vi "MQTT Client - Configure Auth.vi"(0 "MQTT Session":T1, 5 "Client ID":string, 7 "Username":string, 9 "Password":string, 11 "error in (no error)":errorcluster) -> (4 "MQTT Session out":T1, 15 "error out":errorcluster)   [LabVIEW 2019, in "KoRE-MQTT.lvlib"]
doc: "<b>Description:</b> This VI configures authentication settings for an MQTT client session. It processes client identification information necessary for establishing user authentication with the MQTT broker.\n\n<b>Input Terminals:</b>\n- <b>MQTT Session [0]</b>: Reference to the MQTT session that will utilize the configured authentication settings.\n- <b>Client ID [5]</b>: Unique identifier for the MQTT client, which establishes its identity when communicating with the broker. A pseudo-random Client ID will be generated if this input terminal is not wired.\n- <b>Username [7]</b>: The username required for authenticating with the MQTT broker. Do not wire this input terminal if you intend to connect anonymously to the MQTT broker but are using this VI to set the Client ID.\n- <b>Password [9]</b>: The password corresponding to the provided username, crucial for the authentication process. This terminal must be wired if the Username terminal is connected.\n\n<b>Output Terminals:</b>\n- <b>MQTT Session out [4]</b>: Reference to the configured MQTT session with the applied authentication settings.\n\n\nCopyright (c) 2025 KoRElibs.com\nSPDX-License-Identifier: EUPL-1.2\n\nThis VI is licensed under the European Union Public License (EUPL) Version 1.2. You may use this VI unmodified in proprietary works. If you distribute a modified version of this file, the modified file must be released under the EUPL-1.2. Full license: https://joinup.ec.europa.eu/asset/eupl/eupl/1.2/"
uses:
  KoRE-MQTT.lvlib
  TypeDefs/MQTT Client Session.ctl
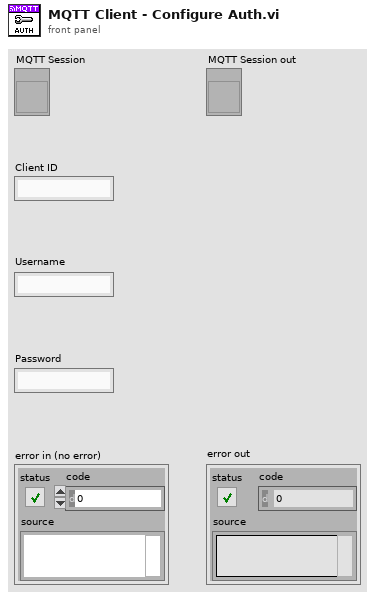
[diagram p1: front panel]
types:
  T1 = typedef "KoRE-MQTT.lvlib/MQTT Client Session.ctl" = refnum<vi>
  T2 = typedef "KoRE-MQTT.lvlib/MQTT Client Session - Data.ctl" = cluster{"TCP ref":refnum<k5>, "Next Packet Id":u16, "Version":u8, "Host":string, "Port":u16, "Ping Delta":u32, "Username":string, "Password":string, "Will QoS":u8, "Will Retain":bool, "Will Topic":string, "Will Payload":string, "TCP Timeout":i32, "Semaphore":T3, "In-Flight Messages":variant, "Close":bool, "Last Send":u32, "Keep Alive":u16, "Last Ping RTT":u32, "Last Ping":u32, "Will Properties":T4[], "Session Expiry Interval":u32, "Maximum QoS":u8, "Retain Available":bool, "Server Maximum Packet Size":u32, "Client Identifier":string, "Server Topic Alias Maximum":u16, "Wildcard Subscription Available":bool, "Subscription Identifier Available":bool, "Shared Subscription Available":bool, "Connect Properties":T5[], "Client Maximum Packet Size":u32, "Client Topic Alias Maximum":u16, "Server Receive Maximum":u16, "Client Receive Maximum":u16, "TLS cfg":refnum<k36>, "Subscriptions":T6[]}
  T3 = typedef "Semaphore RefNum" = refnum<k1>
  T4 = typedef "KoRE-MQTT.lvlib/MQTT Property - Will.ctl" = cluster{"Property":u8, "Value":string}
  T5 = typedef "KoRE-MQTT.lvlib/MQTT Property - CONNECT.ctl" = cluster{"Property":u8, "Value":string}
  T6 = typedef "KoRE-MQTT.lvlib/MQTT Subscription - Info.ctl" = cluster{"Packet Id":u16, "Index":u16, "Identifier":u32, "QoS":u8, "Topic Filter":string, "Reason Code":u8, "Reason String":string, "Granted":bool}
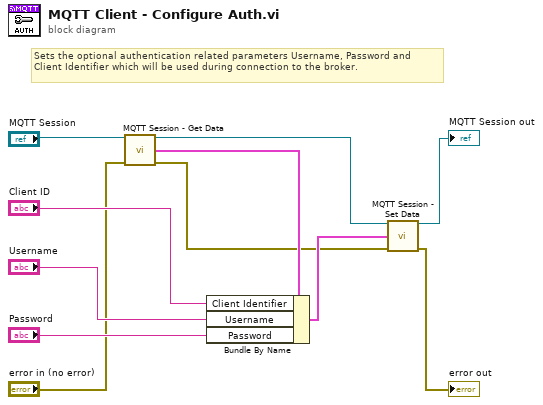
[diagram p0: block diagram]
diagram:
  # "Sets the optional authentication related parameters Username, Password and Client Identifier which will be used during connection to the broker."
  n1 = call "MQTT Session - Get Data.vi"("mqtt ref in"="MQTT Session", "error in"="error in (no error)") -> ("mqtt ref out"=w8:T1, "mqtt ref data"=w6:T2, "error out"=w2:errorcluster)  [unwired: 11 in]
  n2 = Bundle By Name(cluster=w6, "Client Identifier"="Client ID", "Username"="Username", "Password"="Password") -> (w5:T2)
  n3 = call "MQTT Session - Set Data.vi"("mqtt ref in"=w8, "mqtt ref data"=w5, "error in"=w2) -> ("mqtt ref out"=→"MQTT Session out":T1, "error out"=→"error out":errorcluster)  [unwired: 11 in]
